vi "Magic.vi"(8 "error in":errorcluster, 9 "Target Path":path, 10 "Target reference":refnum<vi>, 11 "Parent ref":refnum<vi>) -> (0 "error out":errorcluster)   [LabVIEW 2019]
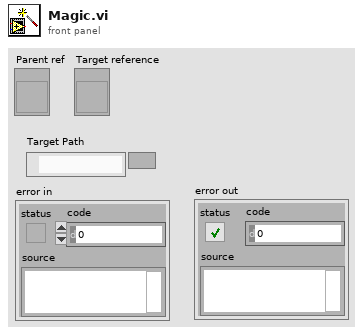
[diagram p1: front panel]
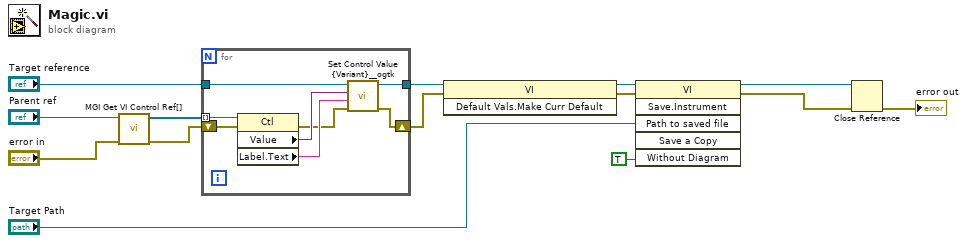
[diagram p0: block diagram]
diagram:
  n1 = call <userlib>:"MGI Get VI Control Ref[].vi"("error in"="error in", "VI (Caller)"="Parent ref") -> ("error out"=w6:errorcluster, "Control[i]"=w13:refnum<vi>[])  [unwired: 6 in, 2 out]
  n2 = for {
    tunnel: w13 -> [w22] mode=indexing
    shift-right: [w15] -> w5
    shift-left: w6 -> [w17]
    tunnel: "Target reference" -> [w19]
    tunnel: [w18] -> w2
    n3 = property class="Ctl"(reference=w22, error in=w17) -> (error out=w16:errorcluster, "Value"=w21:variant, "Label.Text"=w20:string)  [unwired: 1 out]
    n4 = call <userlib>:"Set Control Value {Variant}__ogtk.vi"("error in (no error)"=w16, "Control Name (\"\": use variant name)"=w20, "Value"=w21, "VI Refnum"=w19) -> ("error out"=w15:errorcluster, "VI Refnum dup"=w18:refnum<vi>)  [unwired: 6 in]
  }
  n5 = invoke class="VI" method="Default Vals.Make Curr Default"(reference=w2, error in=w5) -> (reference out=w11:refnum<vi>, error out=w7:errorcluster)  [unwired: 1 in, 1 out]
  n6 = invoke class="VI" method="Save.Instrument"(reference=w11, error in=w7, "Path to saved file"="Target Path", "Without Diagram"=TRUE) -> (reference out=w8:refnum<vi>, error out=w1:errorcluster)  [unwired: 2 in, 4 out]
  n7 = Close Reference(reference=w8, error in (no error)=w1) -> (error out=→"error out":errorcluster)
